vi "CSM - Make String Arguments Safe.vi"(2 "Argument String":string="eaasdf->fqwvrf", 4 "Ignore Argument Type(F)":bool) -> (7 "Safe Argument String":string)   [LabVIEW 2017, in "Communicable State Machine.lvlib"]
doc: "Converts CSM keywords in the argument string to %Hex format to ensure that CSM message string parsing is not affected.\n\n\n> [!NOTE] <b>CSM Message Keywords</b>\n>\n> The following are CSM message keywords: `->`, `->|`, `-@`, `-&`, `<-`, `\\r`, `\\n`, `//`, `>>`, `>>>`, `>>>>`, `;`, `,`.\n\n\n> [!NOTE] <b>CSM Safe String Argument</b>\n>\n> To pass arbitrary strings in CSM arguments without disrupting message parsing, CSM has a built-in Safe-String encoding/decoding scheme. The argument type string is SAFESTR. The conversion process is as follows:\n> 1. Scan the input string. If any CSM keywords, such as `->`, `;`, `\\r` appear, replace them with `%Hex` escape sequences.\n> 2. Obtain the argument in the form `<SAFESTR> escaped string`, which can be safely embedded in the state string without disrupting CSM message parsing.\n\n\n<b>Reference Example</b>: `[CSM-Example]\\0. Base Concepts\\4.3 Arguments - Safe Arguments if it contains key words of CSM.vi`.\n\n-- <b>Controls</b> --\n- <b>Argument String</b>: String argument.\n- <b>Ignore Argument Type(F)</b>: Do not append argument type `SAFESTR`.\n\n-- <b>Indicators</b> --\n- <b>Safe Argument String</b>: Safe string argument."
uses:
  Communicable State Machine.lvlib
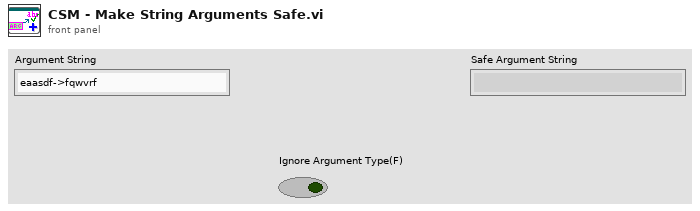
[diagram p1: front panel]
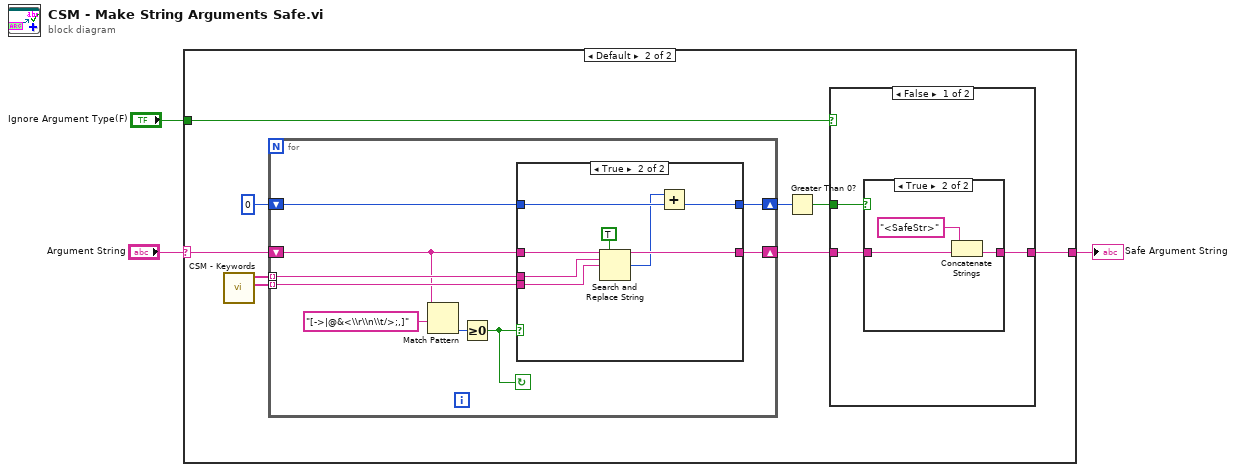
[diagram p0: block diagram]
diagram:
  n1 = case shown="Default" "Argument String" {
    selector: "Argument String" -> [_ w10]
    tunnel: [_ w12] -> w2
    tunnel: "Ignore Argument Type(F)" -> [_ w11]
    frame "" {
    }
    frame Default {
      n2 = call "CSM - Keywords.vi"() -> ("Keywords (%Hex Format)"=w8:string[], "Keywords"=w9:string[])  [unwired: 10 in]
      n3 = for {
        shift-right: [w29] -> w7
        shift-left: w10 -> [w22]
        tunnel: w8 -> [w27] mode=indexing
        tunnel: w9 -> [w28] mode=indexing
        shift-right: [w25] -> w5
        shift-left: 0 -> [w26]
        stop <- w21 continue-if-true
        n4 = Match Pattern(string=w22, regular expression="[->|@&<\\r\\n\\t/>;,]") -> (offset past match=w24:i32)  [unwired: 1 in, 3 out]
        n5 = Greater Or Equal To 0?(x=w24) -> (x >= 0?=w21:bool)
        n6 = case shown="True" w21 {
          tunnel: [w30 w38] -> w29
          tunnel: w28 -> [_ w37]
          tunnel: w27 -> [_ w36]
          tunnel: w26 -> [w31 w35]
          tunnel: [w31 w34] -> w25
          tunnel: w22 -> [w30 w32]
          frame False {
          }
          frame True {
            n7 = Search and Replace String(replace all?=TRUE ("replace all? (F)"), input string=w32, search string=w37, replace string=w36) -> (result string=w38:string, number of replacements=w33:i32)  [unwired: 4 in, 2 out]
            n8 = Add(x=w33, y=w35) -> (x+y=w34:i32)
          }
        }
      }
      n9 = Greater Than 0?(x=w5) -> (x > 0?=w4:bool)
      n10 = case shown="False" w11 {
        tunnel: w7 -> [w15 w20]
        tunnel: [w14 w20] -> w12
        tunnel: w4 -> [w13 _]
        frame False {
          n11 = case shown="True" w13 {
            tunnel: w15 -> [w16 w18]
            tunnel: [w16 w17] -> w14
            frame False {
            }
            frame True {
              n12 = Concatenate Strings("<SafeStr>" ("string"), w18) -> (w17:string)
            }
          }
        }
        frame True {
        }
      }
    }
  }
  "Safe Argument String" <- w2
